vi "FlatToRichauth_LogoutResponse.vi"(5 "OutputClusterType":T1, 11 "InputCluster":T2) -> (3 "OutputCluster":T1)   [LabVIEW 2020, in "grpc-auth_client.lvlib"]
uses:
  grpc-auth_client.lvlib
  auth_LogoutResponse_Flat.ctl
  auth_LogoutResponse.ctl
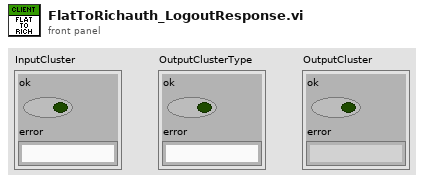
[diagram p1: front panel]
types:
  T1 = typedef "grpc-auth_client.lvlib/auth_LogoutResponse.ctl" = cluster{"ok":bool, "error":string}
  T2 = typedef "grpc-auth_client.lvlib/auth_LogoutResponse_Flat.ctl" = cluster{"ok":bool, "error":string}
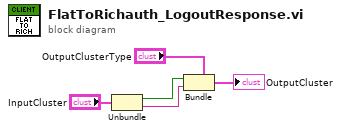
[diagram p0: block diagram]
diagram:
  n1 = Unbundle "Unbundle"("InputCluster") -> ("ok"=w2:bool, "error"=w1:string)
  n2 = Bundle "Bundle"(cluster="OutputClusterType", "ok"=w2, "error"=w1) -> (→"OutputCluster":T1)
